vi "Open File for Writing.vi"(8 "error in (no error)":errorcluster, 11 "Configuration File in":refnum<class "Configuration File.lvclass">) -> (0 "error out":errorcluster, 1 "File was Open?":bool, 2 "refnum out":T2, 3 "Configuration File out":refnum<class "Configuration File.lvclass">, 5 "semaphore":T1)   [LabVIEW 2020, in "Configuration File.lvclass"]
doc: "The purpose of this VI is to prevent race conditions when references to files are opened in from many locations."
uses:
  Configuration File.lvclass
  C:/Git/astemes-triarc-framework/source/Framework/Configuration/Configuration.lvclass
  <vilib>/Utility/config.llb/Config Data RefNum.ctl
  Base/Base.lvclass/Base.ctl
  Configuration/Protected/Get Config Ref.vi
  <vilib>/Utility/error.llb/Clear Errors.vi
  Base/Public/Read Config File Path.vi
  Base/Base.lvclass
  <vilib>/Utility/config.llb/NI_LVConfig.lvlib
  <vilib>/ErrorRing/Error Ring.xnode
  <vilib>/Utility/error.llb/Error Cluster From Error Code.vi
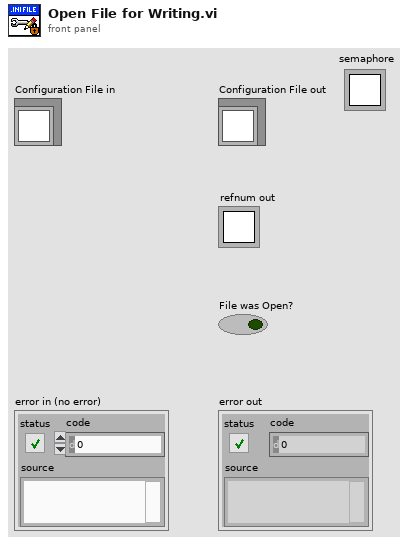
[diagram p1: front panel]
types:
  T1 = typedef "Semaphore RefNum" = refnum<k1>
  T2 = typedef "NI_LVConfig.lvlib/Config Data RefNum.ctl" = refnum<k1>
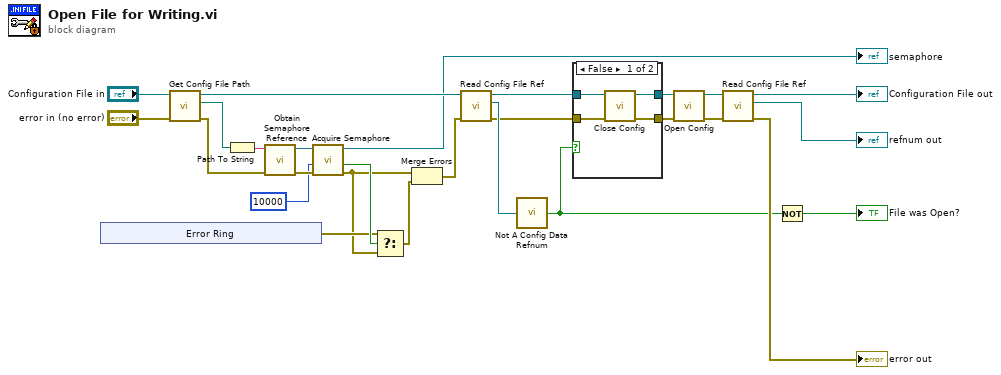
[diagram p0: block diagram]
diagram:
  n1 = xnode "Error Ring"() -> ("error out"=w4:errorcluster)
  n2 = call "Get Config File Path.vi"("error in (no error)"="error in (no error)", "Configuration File In"="Configuration File in") -> ("error out"=w12:errorcluster, "Config File Path"=w11:path, "Configuration File Out"=w14:refnum<class "Configuration File.lvclass">)  [unwired: 7 in]
  n3 = Path To String(path=w11) -> (string=w10:string)
  n4 = call <vilib>:"Obtain Semaphore Reference.vi"("error in (no error)"=w12, "name (unnamed)"=w10) -> ("error out"=w9:errorcluster, "semaphore"=w8:T1)  [unwired: 3 in, 1 out]
  n5 = call <vilib>:"Acquire Semaphore.vi"("error in (no error)"=w9, "ms timeout (-1)"=10000, "semaphore"=w8) -> ("error out"=w3:errorcluster, "timed out"=w5:bool, "semaphore out"=→"semaphore":T1)  [unwired: 2 in]
  n6 = Select(t=w4, s=w5, f=w3) -> (s? t:f=w1:errorcluster)
  n7 = Merge Errors(w3, w1) -> (w2:errorcluster)
  n8 = call "Read Config File Ref.vi"("error in (no error)"=w2, "Configuration File In"=w14) -> ("error out"=w26:errorcluster, "refnum out"=w27:T2, "Configuration File Out"=w25:refnum<class "Configuration File.lvclass">)  [unwired: 7 in]
  n9 = call <vilib>:"Not A Config Data Refnum.vi"("refnum"=w27) -> ("not a config data refnum"=w16:bool)
  n10 = case shown="False" w16 {
    tunnel: w26 -> [w31 w32]
    tunnel: w25 -> [w30 w33]
    tunnel: [w29 w33] -> w19
    tunnel: [w28 w32] -> w18
    frame False {
      n11 = call-dynamic "Close Config.vi"("error in (no error)"=w31, "Configuration File File In"=w30) -> ("error out"=w28:errorcluster, "Configuration File File Out"=w29:refnum<class "Configuration File.lvclass">)  [unwired: 8 in]
    }
    frame True {
    }
  }
  n12 = call-dynamic "Open Config.vi"("error in (no error)"=w18, "Configuration File File In"=w19) -> ("error out"=w23:errorcluster, "Configuration File File Out"=w20:refnum<class "Configuration File.lvclass">)  [unwired: 8 in]
  n13 = call "Read Config File Ref.vi"("error in (no error)"=w23, "Configuration File In"=w20) -> ("error out"=→"error out":errorcluster, "refnum out"=→"refnum out":T2, "Configuration File Out"=→"Configuration File out":refnum<class "Configuration File.lvclass">)  [unwired: 7 in]
  n14 = Not(x=w16) -> (.not. x?=→"File was Open?":bool)
